vi "2.Option_window.vi"(8 "error in (no error) 2":errorcluster) -> (0 "error in (no error) 3":errorcluster)   [LabVIEW 2021]
uses:
  controls/Option_Window.ctl
  Control/Ini.ctl
  Control/Set_Get.ctl
  Control/Mode.ctl
  controls/test_sequence .ctl
panel:
  in  "Remove User":bool
  out "Back Button 2":bool
  in  "Back Button":bool
  in  "Tab Control":T1(tab)
  in  "Mode":bool
  in  "Select Button":bool
  in  "Create User":bool
  in  "Test":bool
  in  "Test Procedure":bool
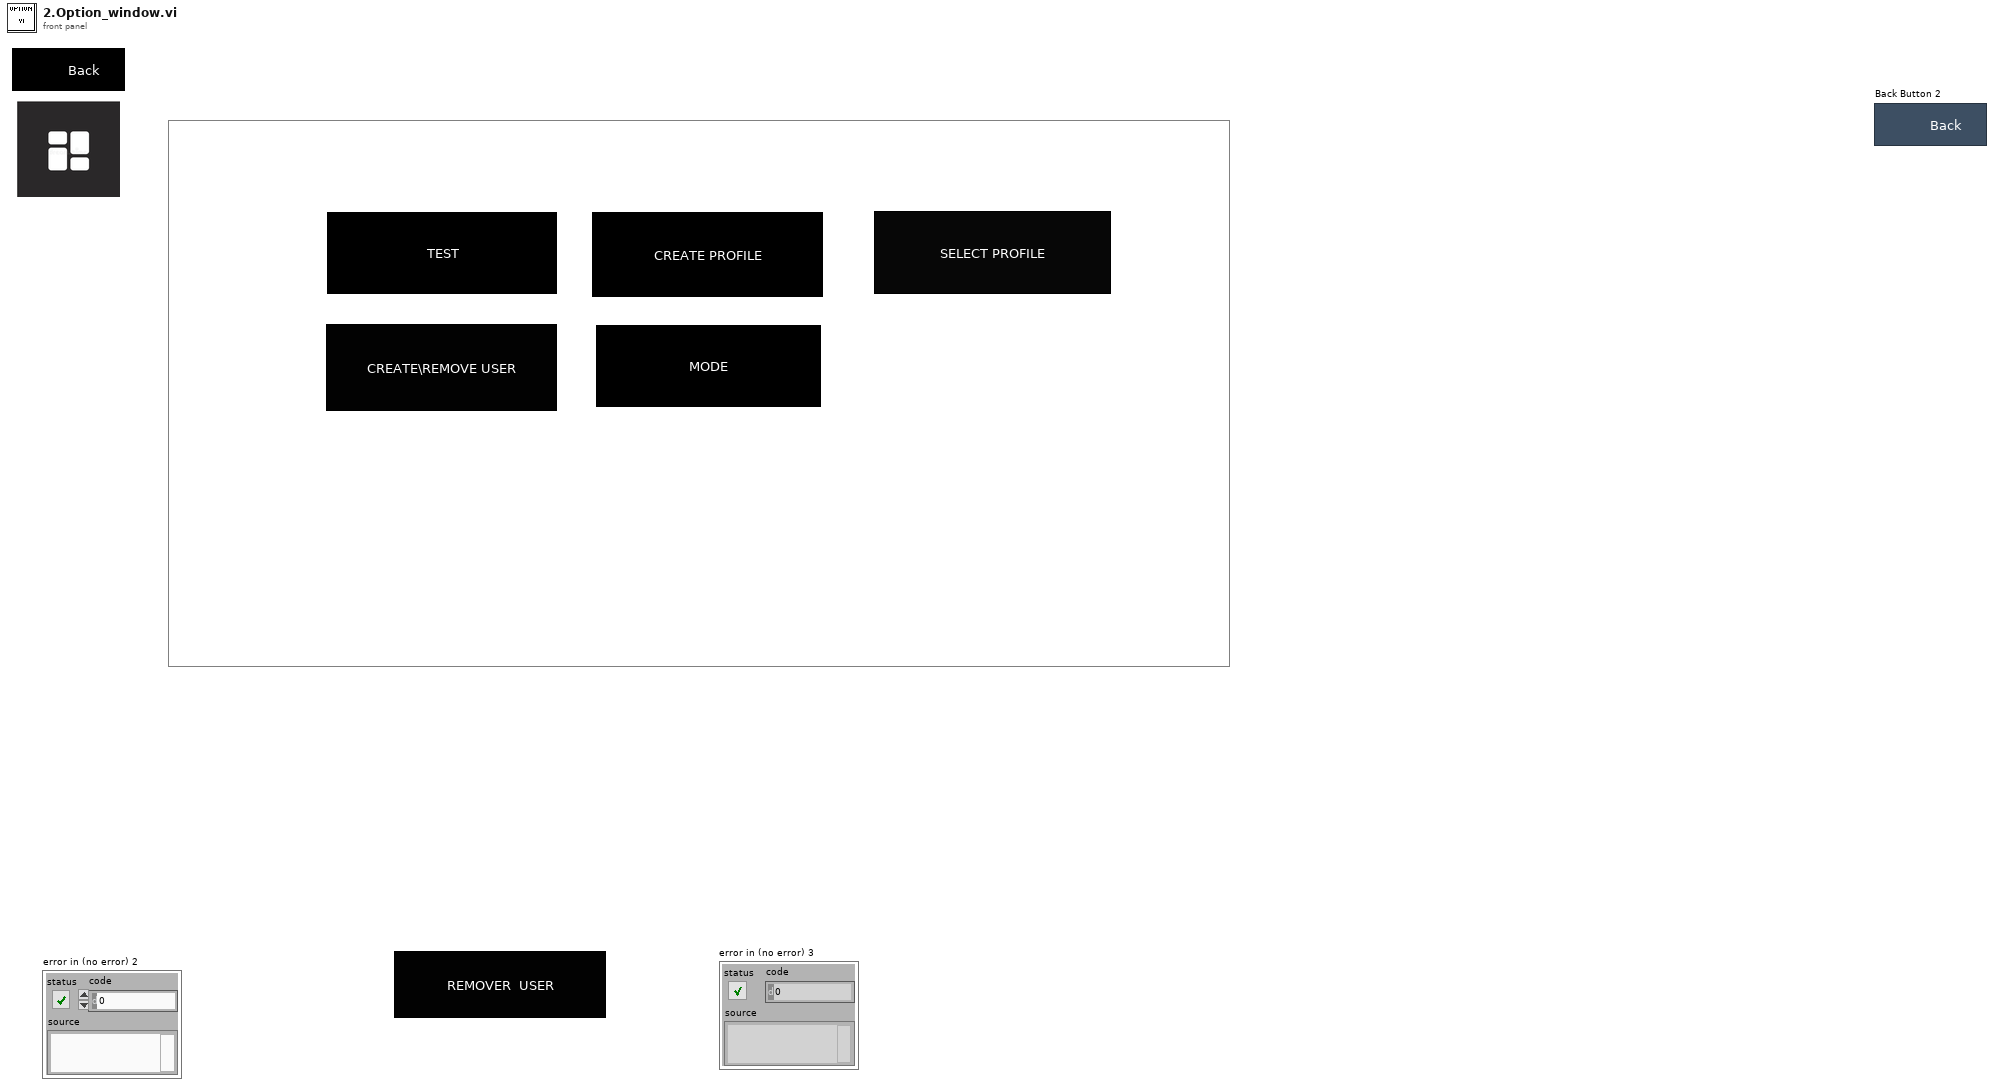
[diagram p1: front panel]
types:
  T1 = enum32{"INITIAL", "TEST PROCEDURE", "USER ACCESS", "ADMIN ACCESS"}
  T2 = typedef "Option_Window.ctl" = enum16{"Initial", "Test Procedure", "User Access", "Admin access", "Add User", "Remover User", "Mode", "Test", "Exit"}
  T3 = typedef "Ini.ctl" = enum16{"Write", "Read"}
  T4 = enum8{"Enabled", "Disabled", "Disabled and Grayed Out"}
  T5 = typedef "Mode.ctl" = enum16{"Offline", "Online"}
  T6 = typedef "Set_Get.ctl" = enum16{"Set", "Get"}
  T7 = typedef "test_sequence .ctl" = enum16{"Init Devices", "Login", "Option Window", "Idle state", "Check", "Uncheck", "Scan Barcode", "Clear the test Containers", "Init-Pre Test", "Test ", "Result", "Report", "Database", "Update Display", "Confirm Quit", "Error", "Exit"}
  T8 = enum32{"INITIAL", "TEST PROCEDURE", "USER ACCESS"}
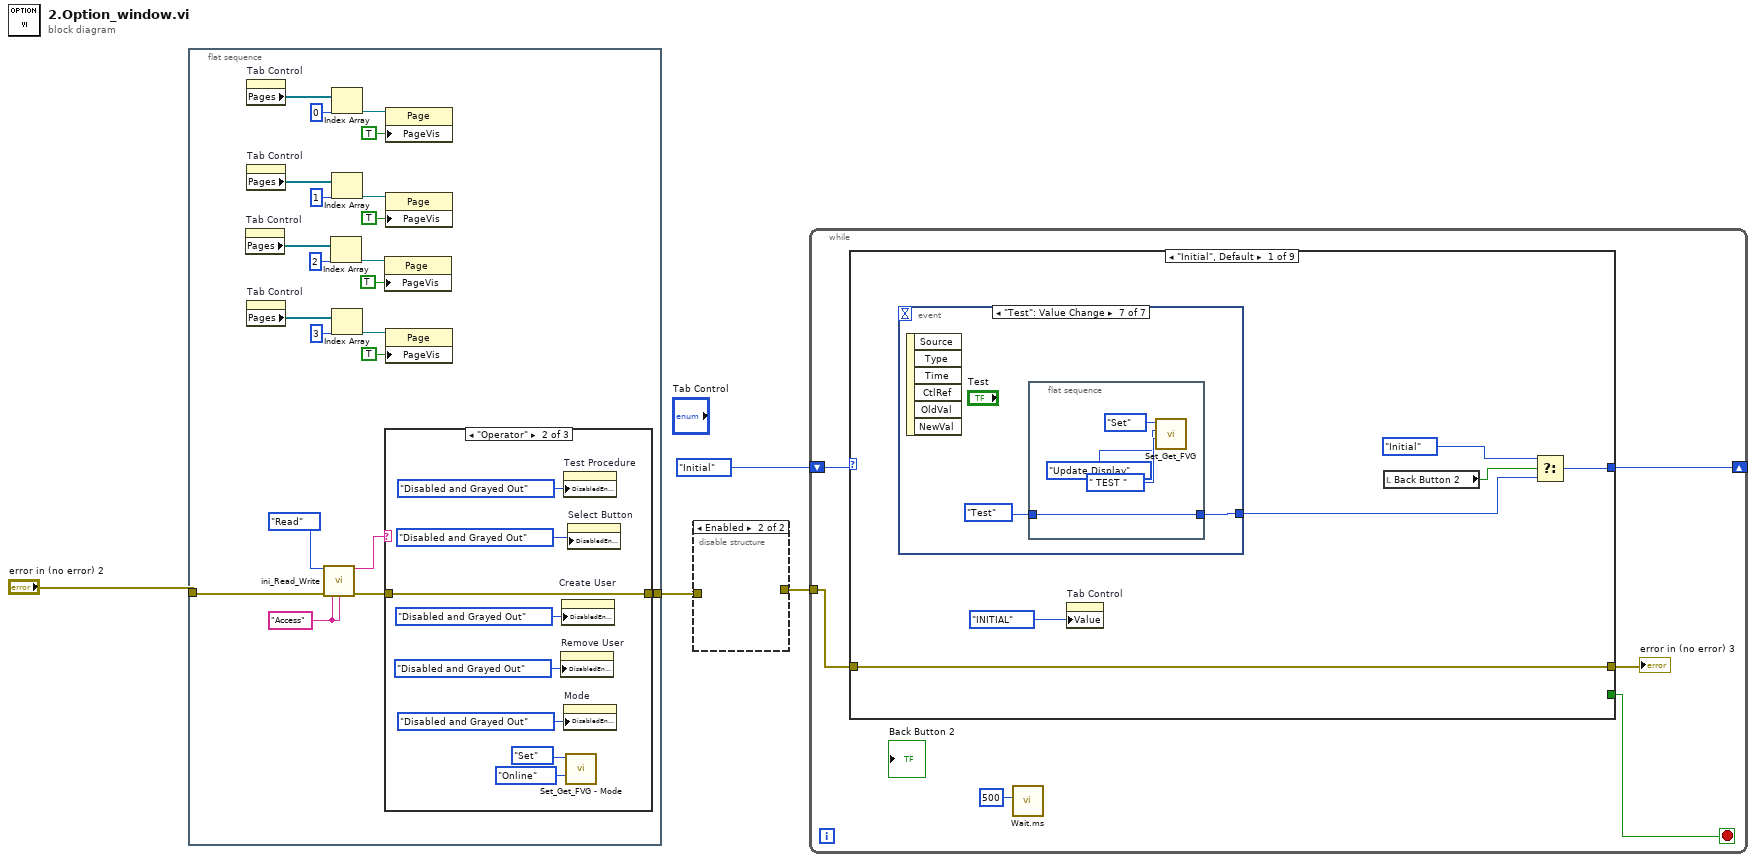
[diagram p0: block diagram]
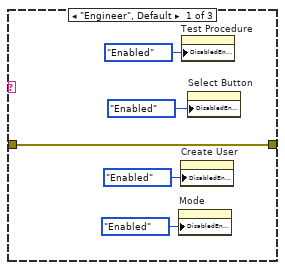
[diagram p3: hidden frame]
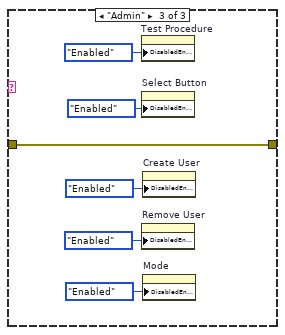
[diagram p4: hidden frame]
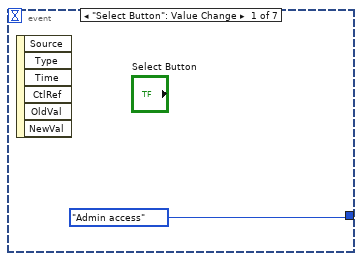
[diagram p5: hidden frame]
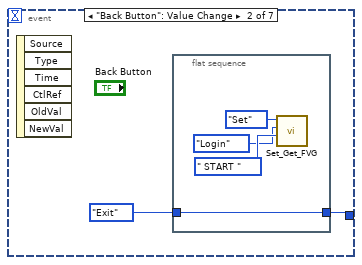
[diagram p6: hidden frame]
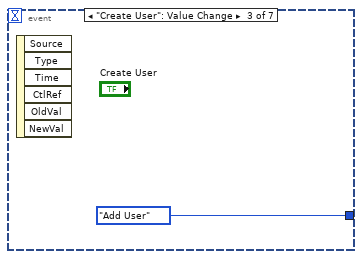
[diagram p7: hidden frame]
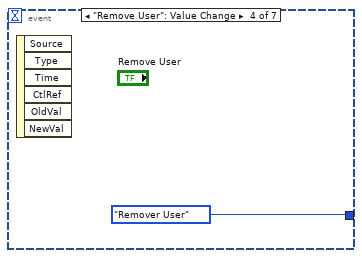
[diagram p8: hidden frame]
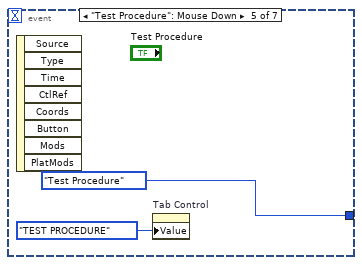
[diagram p9: hidden frame]
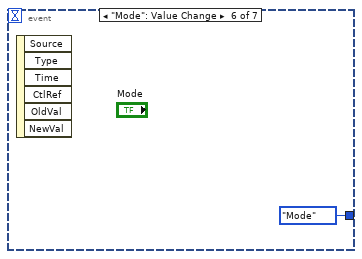
[diagram p10: hidden frame]
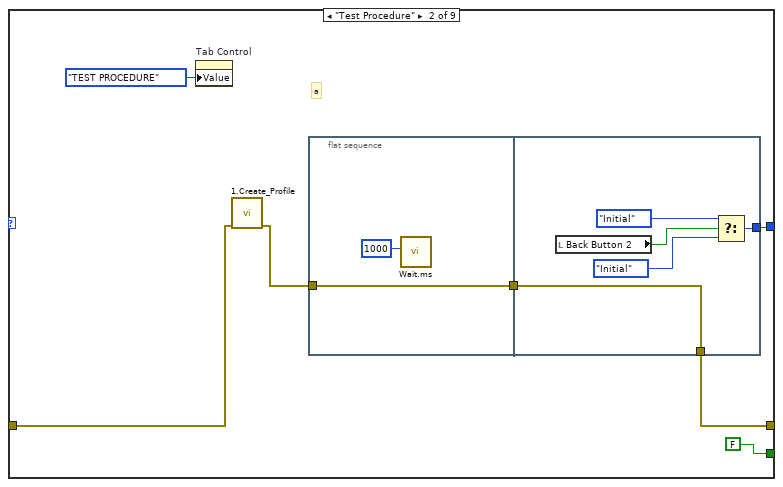
[diagram p11: hidden frame]
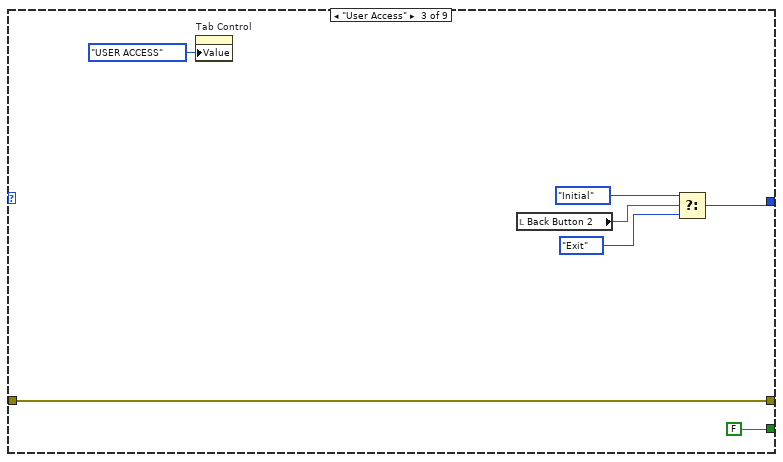
[diagram p12: hidden frame]
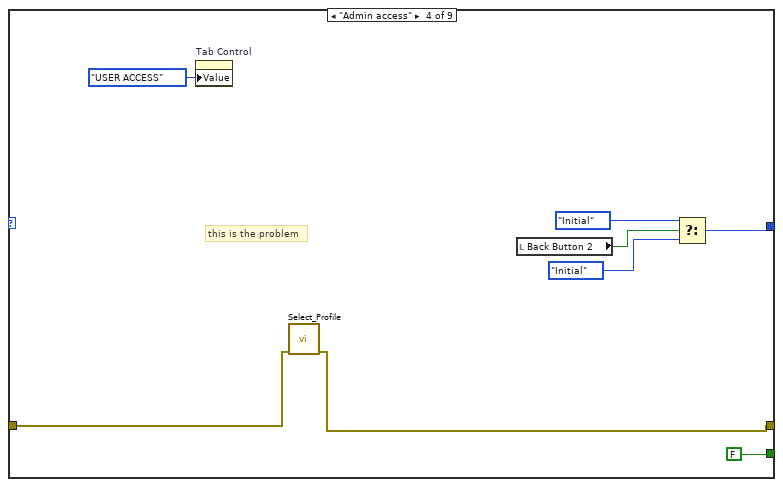
[diagram p13: hidden frame]
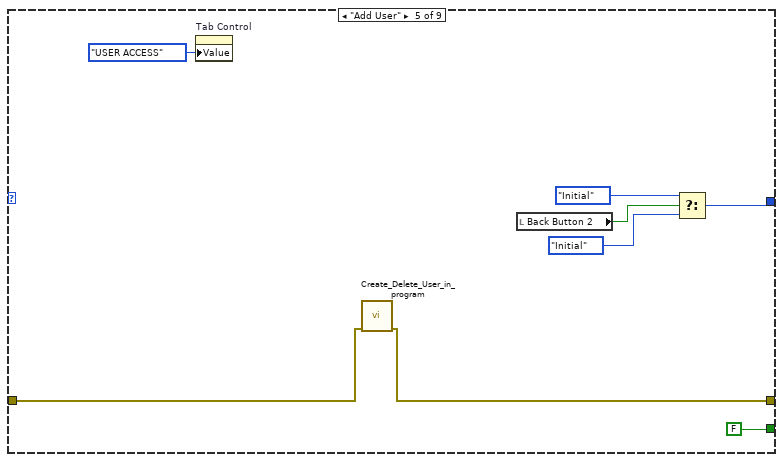
[diagram p14: hidden frame]
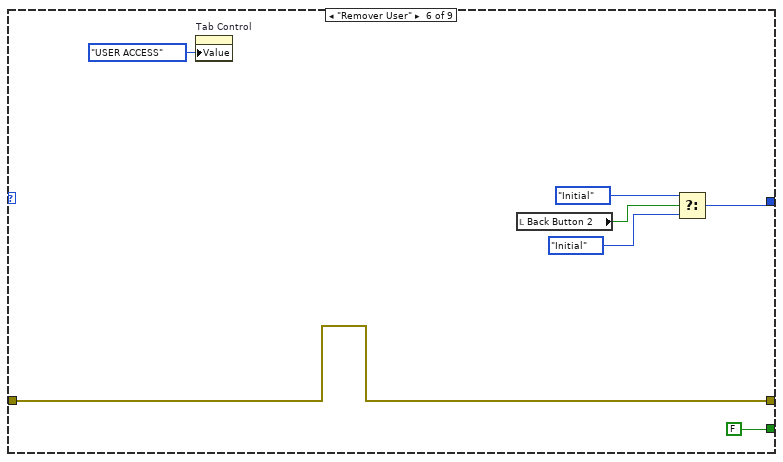
[diagram p15: hidden frame]
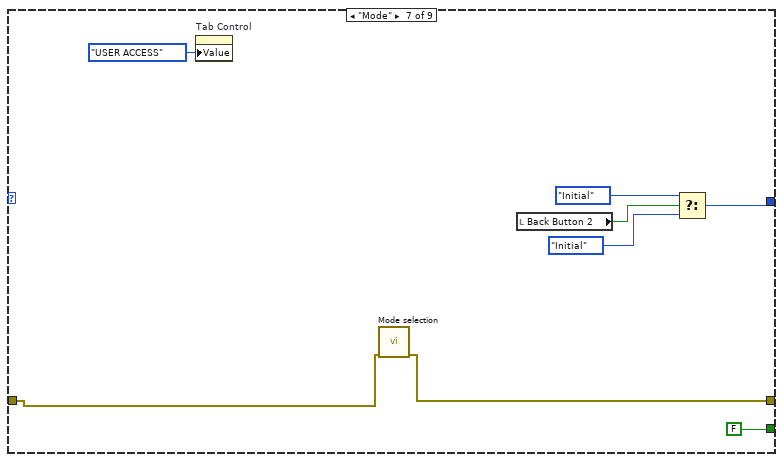
[diagram p16: hidden frame]
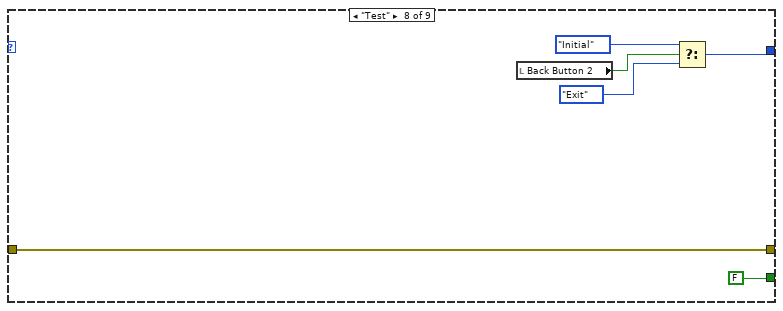
[diagram p17: hidden frame]
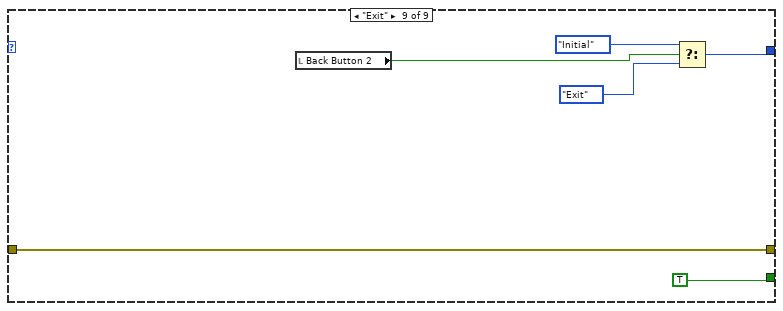
[diagram p18: hidden frame]
diagram:
  n1 = flat-sequence {
    tunnel: "error in (no error) 2" -> [w26]
    tunnel: [w22] -> w2
    frame #0 {
      w5 = "Access" ("Read")
      n2 = property on="Tab Control" class="TabCtl (strict)"() -> ("Pages"=w13:refnum<vi>[])  [unwired: 2 in, 2 out]
      n3 = property on="Tab Control" class="TabCtl (strict)"() -> ("Pages"=w17:refnum<vi>[])  [unwired: 2 in, 2 out]
      n4 = property on="Tab Control" class="TabCtl (strict)"() -> ("Pages"=w18:refnum<vi>[])  [unwired: 2 in, 2 out]
      n5 = property on="Tab Control" class="TabCtl (strict)"() -> ("Pages"=w6:refnum<vi>[])  [unwired: 2 in, 2 out]
      n6 = call "ini_Read_Write.vi"(0:Ini."Read", "error in (no error) 2"=w26, "Read Section"=w5, "Read Key"=w5) -> ("value"=w24:string, "error in (no error) 3"=w23:errorcluster)  [unwired: 10 in]
      n7 = Index Array(array=w13, index=2) -> (element=w10:refnum<vi>)
      n8 = Index Array(array=w17, index=0) -> (element=w14:refnum<vi>)
      n9 = Index Array(array=w18, index=1) -> (element=w21:refnum<vi>)
      n10 = Index Array(array=w6, index=3) -> (element=w9:refnum<vi>)
      n11 = property class="Page"(reference=w10, "PageVis"=TRUE ("Page Visible")) -> ()  [unwired: 1 in, 2 out]
      n12 = case shown="\"Operator\"" w24 {
        tunnel: w23 -> [w31 w39 w45]
        tunnel: [w31 w39 w45] -> w22
        frame "Engineer", Default {
          n13 = property on="Mode" class="Bool"("DisabledEnum"=T4."Enabled" ("Disabled")) -> ()  [unwired: 2 in, 2 out]
          n14 = property on="Create User" class="Bool"("DisabledEnum"=T4."Enabled" ("Disabled")) -> ()  [unwired: 2 in, 2 out]
          n15 = property on="Test Procedure" class="Bool"("DisabledEnum"=T4."Enabled" ("Disabled")) -> ()  [unwired: 2 in, 2 out]
          n16 = property on="Select Button" class="Bool"("DisabledEnum"=T4."Enabled" ("Disabled")) -> ()  [unwired: 2 in, 2 out]
        }
        frame "Operator" {
          n17 = property on="Remove User" class="Bool"("DisabledEnum"=T4."Disabled and Grayed Out" ("Disabled")) -> ()  [unwired: 2 in, 2 out]
          n18 = property on="Create User" class="Bool"("DisabledEnum"=T4."Disabled and Grayed Out" ("Disabled")) -> ()  [unwired: 2 in, 2 out]
          n19 = property on="Test Procedure" class="Bool"("DisabledEnum"=T4."Disabled and Grayed Out" ("Disabled")) -> ()  [unwired: 2 in, 2 out]
          n20 = property on="Mode" class="Bool"("DisabledEnum"=T4."Disabled and Grayed Out" ("Disabled")) -> ()  [unwired: 2 in, 2 out]
          n21 = call "Set_Get_FVG - Mode.vi"(10:Mode."Online", "Enum"=Set_Get."Set") -> ()  [unwired: 8 in, 2 out]
          n22 = property on="Select Button" class="Bool"("DisabledEnum"=T4."Disabled and Grayed Out" ("Disabled")) -> ()  [unwired: 2 in, 2 out]
        }
        frame "Admin" {
          n23 = property on="Test Procedure" class="Bool"("DisabledEnum"=T4."Enabled" ("Disabled")) -> ()  [unwired: 2 in, 2 out]
          n24 = property on="Select Button" class="Bool"("DisabledEnum"=T4."Enabled" ("Disabled")) -> ()  [unwired: 2 in, 2 out]
          n25 = property on="Remove User" class="Bool"("DisabledEnum"=T4."Enabled" ("Disabled")) -> ()  [unwired: 2 in, 2 out]
          n26 = property on="Create User" class="Bool"("DisabledEnum"=T4."Enabled" ("Disabled")) -> ()  [unwired: 2 in, 2 out]
          n27 = property on="Mode" class="Bool"("DisabledEnum"=T4."Enabled" ("Disabled")) -> ()  [unwired: 2 in, 2 out]
        }
      }
      n28 = property class="Page"(reference=w14, "PageVis"=TRUE ("Page Visible")) -> ()  [unwired: 1 in, 2 out]
      n29 = property class="Page"(reference=w21, "PageVis"=TRUE ("Page Visible")) -> ()  [unwired: 1 in, 2 out]
      n30 = property class="Page"(reference=w9, "PageVis"=TRUE ("Page Visible")) -> ()  [unwired: 1 in, 2 out]
    }
  }
  n31 = disable-structure shown="Enabled" {
    disable-tunnel: w2 -> [w46 _]
    disable-tunnel: [w46 _] -> w1
    frame Disabled {
    }
    frame Enabled {
    }
  }
  n32 = while {
    shift-right: [w51] -> _
    shift-left: Option_Window."Initial" -> [w52]
    tunnel: w1 -> [w50]
    stop <- w47 stop-if-true
    n33 = case shown="\"Initial\", Default" w52 {
      tunnel: [w58 w83 w97 w105 w113 w120 w128 w134 w140] -> w51
      tunnel: [_ FALSE FALSE FALSE FALSE FALSE FALSE FALSE TRUE] -> w47
      tunnel: w50 -> [w54 w77 w91 w99 w106 w114 w122 w129 w135]
      tunnel: [w54 w79 w91 w98 w107 w114 w121 w129 w135] -> w49
      frame "Initial", Default {
        n34 = event shown="[6] \"Test\": Value Change" {
          selector: _ -> [_ _ _ _ _ _ _]
          dyn-events: _ -> [_ _ _ _ _ _ _]
          timeout: _ -> [_ _ _ _ _ _ _]
          tunnel: [Option_Window."Admin access" w60 Option_Window."Add User" Option_Window."Remover User" Option_Window."Test Procedure" Option_Window."Mode" w71] -> w55
          event "Select Button": Value Change {
            n35 = event-data() -> ()  [unwired: 1 in, 6 out]
          }
          event "Back Button": Value Change {
            n36 = event-data() -> ()  [unwired: 1 in, 6 out]
            n37 = flat-sequence {
              tunnel: Option_Window."Exit" -> [w64]
              tunnel: [w64] -> w60
              frame #0 {
                n38 = call "Set_Get_FVG.vi"("Tab Control"=enum32{" START ", " HOME ", " TEST "}." START ", "Message"=test_sequence_."Login", "Enum"=Set_Get."Set") -> ()  [unwired: 6 in, 3 out]
              }
            }
          }
          event "Create User": Value Change {
            n39 = event-data() -> ()  [unwired: 1 in, 6 out]
          }
          event "Remove User": Value Change {
            n40 = event-data() -> ()  [unwired: 1 in, 6 out]
          }
          event "Test Procedure": Mouse Down {
            n41 = event-data() -> ()  [unwired: 1 in, 8 out]
            n42 = property on="Tab Control" class="TabCtl (strict)"("Value"=enum32{"INITIAL", "TEST PROCEDURE"}."TEST PROCEDURE" ("Tab Control")) -> ()  [unwired: 2 in, 2 out]
          }
          event "Mode": Value Change {
            n43 = event-data() -> ()  [unwired: 1 in, 6 out]
          }
          event "Test": Value Change {
            n44 = event-data() -> ()  [unwired: 1 in, 6 out]
            n45 = flat-sequence {
              tunnel: Option_Window."Test" -> [w76]
              tunnel: [w76] -> w71
              frame #0 {
                n46 = call "Set_Get_FVG.vi"("Tab Control"=enum32{" START ", " HOME ", " TEST "}." TEST ", "Message"=test_sequence_."Update Display", "Enum"=Set_Get."Set") -> ()  [unwired: 6 in, 3 out]
              }
            }
          }
        }
        n47 = property on="Tab Control" class="TabCtl (strict)"("Value"=enum32{"INITIAL", "TEST PROCEDURE"}."INITIAL" ("Tab Control")) -> ()  [unwired: 2 in, 2 out]
        n48 = local read "Back Button 2"() -> (w57:bool)
        n49 = Select(t=Option_Window."Initial" ("f"), s=w57, f=w55) -> (s? t:f=w58:T2)
      }
      frame "Test Procedure" {
        # "a"
        n50 = property on="Tab Control" class="TabCtl (strict)"("Value"=enum32{"INITIAL", "TEST PROCEDURE"}."TEST PROCEDURE" ("Tab Control")) -> ()  [unwired: 2 in, 2 out]
        n51 = call "1.Create_Profile.vi"("error out"=w77) -> ("error out"=w78:errorcluster)  [unwired: 10 in]
        n52 = flat-sequence {
          tunnel: w78 -> [w84]
          tunnel: [w84] -> w80
          tunnel: [w90] -> w83
          tunnel: w80 -> [w86]
          tunnel: [w86] -> w79
          frame #0 {
            n53 = call "Wait.ms.vi"("milliseconds to wait"=u32 1000) -> ()  [unwired: 10 in, 1 out]
          }
          frame #1 {
            n54 = local read "Back Button 2"() -> (w87:bool)
            n55 = Select(t=Option_Window."Initial", s=w87, f=Option_Window."Initial") -> (s? t:f=w90:T2)
          }
        }
      }
      frame "User Access" {
        n56 = property on="Tab Control" class="TabCtl (strict)"("Value"=T8."USER ACCESS" ("Tab Control")) -> ()  [unwired: 2 in, 2 out]
        n57 = local read "Back Button 2"() -> (w93:bool)
        n58 = Select(t=Option_Window."Initial", s=w93, f=Option_Window."Exit") -> (s? t:f=w97:T2)
      }
      frame "Admin access" {
        # "this is the problem"
        n59 = property on="Tab Control" class="TabCtl (strict)"("Value"=T8."USER ACCESS" ("Tab Control")) -> ()  [unwired: 2 in, 2 out]
        n60 = call "Select_Profile.vi"("error in"=w99) -> ("error out"=w98:errorcluster)  [unwired: 8 in, 1 out]
        n61 = local read "Back Button 2"() -> (w101:bool)
        n62 = Select(t=Option_Window."Initial", s=w101, f=Option_Window."Initial") -> (s? t:f=w105:T2)
      }
      frame "Add User" {
        n63 = property on="Tab Control" class="TabCtl (strict)"("Value"=T8."USER ACCESS" ("Tab Control")) -> ()  [unwired: 2 in, 2 out]
        n64 = call "Create_Delete_User_in_program.vi"("error in (no error) 3"=w106) -> ("error in (no error) 4"=w107:errorcluster)  [unwired: 10 in]
        n65 = local read "Back Button 2"() -> (w109:bool)
        n66 = Select(t=Option_Window."Initial", s=w109, f=Option_Window."Initial") -> (s? t:f=w113:T2)
      }
      frame "Remover User" {
        n67 = property on="Tab Control" class="TabCtl (strict)"("Value"=T8."USER ACCESS" ("Tab Control")) -> ()  [unwired: 2 in, 2 out]
        n68 = local read "Back Button 2"() -> (w116:bool)
        n69 = Select(t=Option_Window."Initial", s=w116, f=Option_Window."Initial") -> (s? t:f=w120:T2)
      }
      frame "Mode" {
        n70 = property on="Tab Control" class="TabCtl (strict)"("Value"=T8."USER ACCESS" ("Tab Control")) -> ()  [unwired: 2 in, 2 out]
        n71 = call "Mode selection .vi"("error out"=w122) -> ("error out 2"=w121:errorcluster)  [unwired: 9 in, 1 out]
        n72 = local read "Back Button 2"() -> (w124:bool)
        n73 = Select(t=Option_Window."Initial", s=w124, f=Option_Window."Initial") -> (s? t:f=w128:T2)
      }
      frame "Test" {
        n74 = local read "Back Button 2"() -> (w131:bool)
        n75 = Select(t=Option_Window."Initial", s=w131, f=Option_Window."Exit") -> (s? t:f=w134:T2)
      }
      frame "Exit" {
        n76 = local read "Back Button 2"() -> (w136:bool)
        n77 = Select(t=Option_Window."Initial", s=w136, f=Option_Window."Exit") -> (s? t:f=w140:T2)
      }
    }
    "error in (no error) 3" <- w49
    n78 = call "Wait.ms.vi"("milliseconds to wait"=u32 500) -> ()  [unwired: 10 in, 1 out]
  }
